vi "Write to All Indicators.vi"(11 "indicator data in":T1[](array[typedef])) -> (0 "errors":errorcluster[](array[cluster]), 3 "indicator data out":T1[](array[typedef]))   [LabVIEW 2018, in "GLog.lvlib" / "UI Updater.lvlib"]
uses:
  UI Updater.lvlib
  Indicator Data.ctl
panel:
  # "Connector Pane"
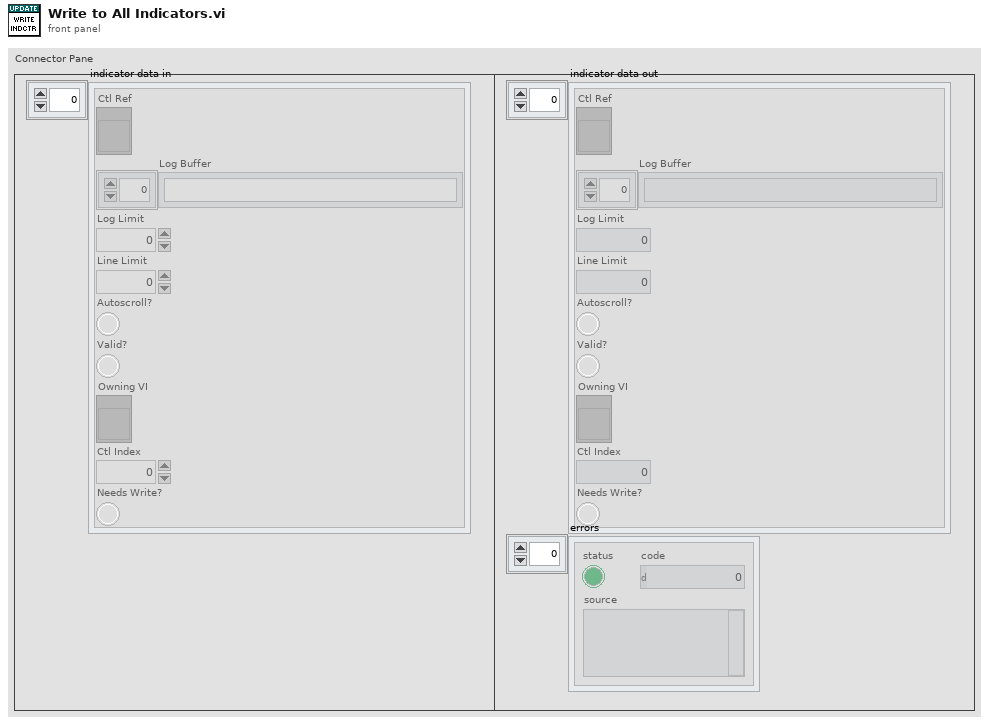
[diagram p1: front panel]
types:
  T1 = typedef "GLog.lvlib/UI Updater.lvlib/Indicator Data.ctl" = cluster{"Ctl Ref":refnum<vi>, "Log Buffer":string[], "Log Limit":i32, "Line Limit":i32, "Autoscroll?":bool, "Valid?":bool, "Owning VI":refnum<vi>, "Ctl Index":i32, "Needs Write?":bool}
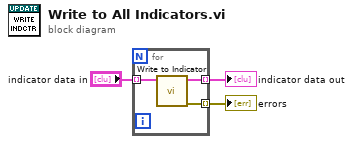
[diagram p0: block diagram]
diagram:
  n1 = for {
    tunnel: "indicator data in" -> [w5] mode=indexing
    tunnel: [w6] -> w2 mode=indexing
    tunnel: [w4] -> w3 mode=indexing
    n2 = call "Write to Indicator.vi"("indicator data in"=w5) -> ("error out"=w6:errorcluster, "indicator data out"=w4:T1)  [unwired: 9 in]
  }
  "indicator data out" <- w3
  "errors" <- w2
